vi "Test Update Account Balance.vi"() -> ()   [LabVIEW 2026]
doc: "Caraya unit test for Update Account Balance.vi (and Read Accounts.vi, which reads the result back). Every case starts from its own fresh copy of the specification accounts file (Create Accounts Fixture.vi, written under Tests\\results), so the real ATM accounts.txt is never touched.\n\nCase 1: setting 45678 to 1000.5 changes exactly that record - all four records are read back and compared, so a corrupted line, a lost record or a rounded balance fails.\nCase 2: an unknown account returns error 5002.\n\nThe error cluster carries the FIRST failure only. Read the JUnit report for all of them."
uses:
  <vilib>/addons/_JKI Toolkits/Caraya/classes/Test/Test.lvclass
  <vilib>/addons/_JKI Toolkits/Caraya/classes/Assert/Assert.lvclass
panel:
  out "error out":errorcluster
  in  "error in":errorcluster
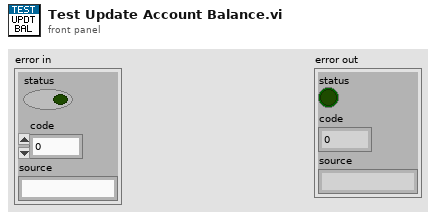
[diagram p1: front panel]
types:
  T1 = cluster{"Account Number":string, "First Name":string, "Last Name":string, "Balance":dbl}[]
  T2 = typedef "ATM Account.ctl" = cluster{"Account Number":string, "First Name":string, "Last Name":string, "Balance":dbl}
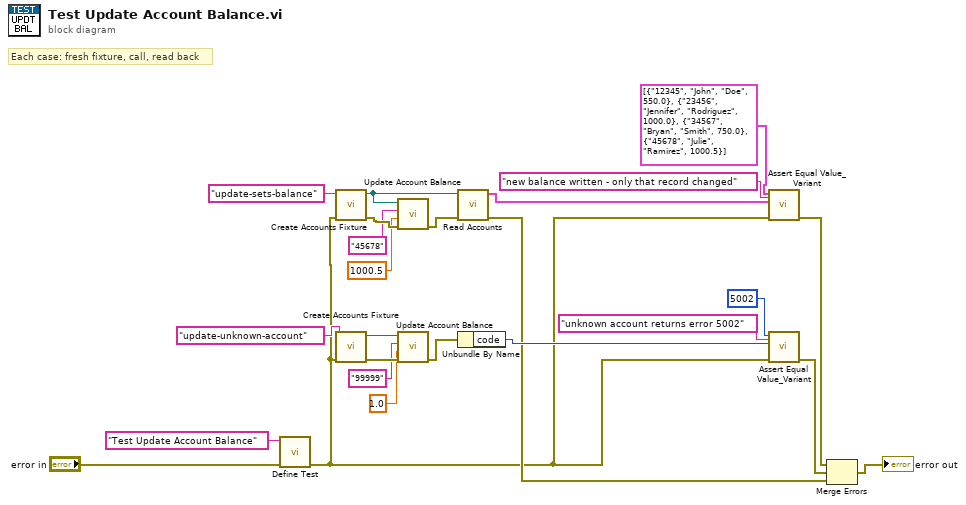
[diagram p0: block diagram]
diagram:
  # "Each case: fresh fixture, call, read back"
  n1 = call <vilib>:"Define Test.vi"("error in (no error)"="error in", "Label (VI Title)"="Test Update Account Balance") -> ("error out"=w4:errorcluster)  [unwired: 8 in, 1 out]
  n2 = call "Create Accounts Fixture.vi"("error in"=w4, "Fixture Name"="update-sets-balance") -> ("error out"=w9:errorcluster, "Accounts File Path"=w8:path)  [unwired: 8 in]
  n3 = call "Create Accounts Fixture.vi"("error in"=w4, "Fixture Name"="update-unknown-account") -> ("error out"=w20:errorcluster, "Accounts File Path"=w19:path)  [unwired: 8 in]
  n4 = call "Update Account Balance.vi"("error in"=w9, "New Balance"=1000.5, "Account Number"="45678", "Accounts File Path"=w8) -> ("error out"=w10:errorcluster)  [unwired: 7 in]
  n5 = call "Update Account Balance.vi"("error in"=w20, "New Balance"=1.0, "Account Number"="99999", "Accounts File Path"=w19) -> ("error out"=w21:errorcluster)  [unwired: 7 in]
  n6 = call "Read Accounts.vi"("error in"=w10, "Accounts File Path"=w8) -> ("error out"=w12:errorcluster, "Accounts"=w11:T2[])  [unwired: 8 in]
  n7 = Unbundle By Name(w21) -> ("code"=w22:i32)
  n8 = call <vilib>:"Assert Equal Value_Variant.vi"("Label"="new balance written - only that record changed", "error in (no error)"=w4, "Actual"=w11, "Expected"=T1 [{"Account Number"="12345", "First Name"="John", "Last Name"="Doe", "Balance"=550.0}, {"Account Number"="23456", "First Name"="Jennifer", "Last Name"="Rodriguez", "Balance"=1000.0}, {"Account Number"="34567", "First Name"="Bryan", "Last Name"="Smith", "Balance"=750.0}, {"Account Number"="45678", "First Name"="Julie", "Last Name"="Ramirez", "Balance"=1000.5}] ("expected 1")) -> ("error out"=w15:errorcluster)  [unwired: 6 in, 1 out]
  n9 = call <vilib>:"Assert Equal Value_Variant.vi"("Label"="unknown account returns error 5002", "error in (no error)"=w4, "Actual"=w22, "Expected"=5002 ("expected 2")) -> ("error out"=w25:errorcluster)  [unwired: 6 in, 1 out]
  n10 = Merge Errors(w15, w25, w12) -> (→"error out":errorcluster)
